vi "Display Client Creation Status.vi"(8 "error in":errorcluster, 9 "client names":string[](array[string]), 10 "status":T1[](array[typedef]), 11 "statusListbox in":refnum<vi>) -> (0 "error out":errorcluster, 2 "all success?":bool, 3 "statusListbox out":refnum<vi>)   [LabVIEW 2021, in "MeasurementClient Editor.lvlib"]
uses:
  MeasurementClient Editor.lvlib
  Client Creation Status.ctl
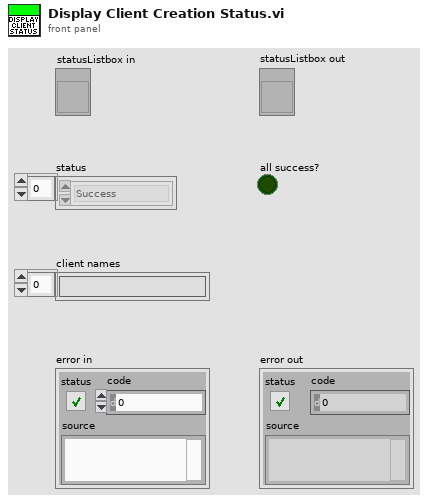
[diagram p1: front panel]
types:
  T1 = typedef "MeasurementClient Editor.lvlib/Client Creation Status.ctl" = enum16{"Success", "Fail"}
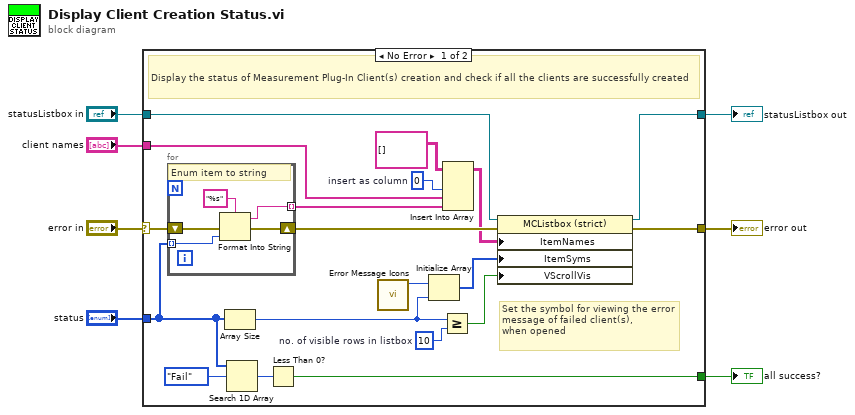
[diagram p0: block diagram]
diagram:
  n1 = case shown="No Error" "error in" {
    selector: "error in" -> [w16 w33]
    tunnel: [w26 _] -> w7
    tunnel: "statusListbox in" -> [w24 w32]
    tunnel: "client names" -> [w10 _]
    tunnel: "status" -> [w14 _]
    tunnel: [w22 w33] -> w2
    tunnel: [w21 w32] -> w1
    frame No Error {
      w11 = 0  # insert as column
      w19 = 10  # no. of visible rows in listbox
      # "Set the symbol for viewing the error message of failed client(s),\nwhen opened"
      # "Display the status of Measurement Plug-In Client(s) creation and check if all the clients are successfully created"
      n2 = for {
        shift-right: [w30] -> w15
        shift-left: w16 -> [w31]
        tunnel: w14 -> [w29] mode=indexing
        tunnel: [w27] -> w9 mode=indexing
        # "Enum item to string"
        n3 = Format Into String(format string="%s", error in=w31, w29) -> (resulting string=w27:string, error out=w30:errorcluster)  [unwired: 1 in]
      }
      n4 = Array Size(array=w14) -> (size(s)=w20:i32)
      n5 = Search 1D Array(1D array=w14, element=Client_Creation_Status."Fail") -> (index of element=w25:i32)  [unwired: 1 in]
      n6 = Less Than 0?(x=w25) -> (x < 0?=w26:bool)
      n7 = call "Error Message Icons.vi"() -> ("closed"=w13:i32)  [unwired: 10 in, 1 out]
      n8 = Initialize Array(w13, w20) -> (w23:i32[])
      n9 = Greater Or Equal?(x=w20, y=w19) -> (x >= y?=w18:bool)
      n10 = Insert Into Array(array=string[][] [], index (col)=w11, new element #1=w10, new element #2=w9) -> (w8:string[][])  [unwired: 1 in]
      n11 = property on="Property Node" class="MCListbox (strict)"(reference=w24, error in=w15, "ItemNames"=w8, "ItemSyms"=w23, "VScrollVis"=w18) -> (reference out=w21:refnum<vi>, error out=w22:errorcluster)
    }
    frame Error {
      # "Pass"
    }
  }
  "all success?" <- w7
  "error out" <- w2
  "statusListbox out" <- w1
